vi "C_CRC32.vi"(8 "error in (no error)":errorcluster, 11 "data":u8[](array[numeric]) format="%.0x") -> (0 "error out":errorcluster, 3 "crc32":u32 format="%.0x")   [LabVIEW 2021, in "CANsub_C.lvlib"]
uses:
  CANsub_C.lvlib
  codec_vis/CANsub_Codec.lvlib
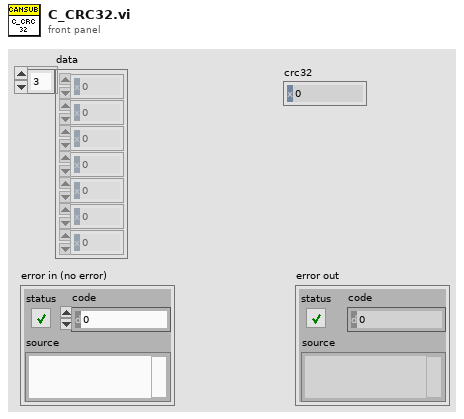
[diagram p1: front panel]
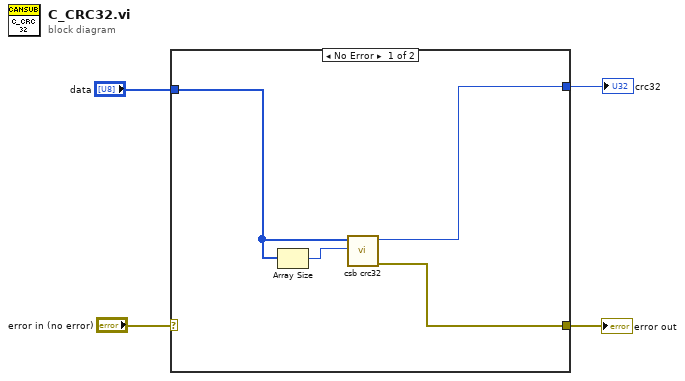
[diagram p0: block diagram]
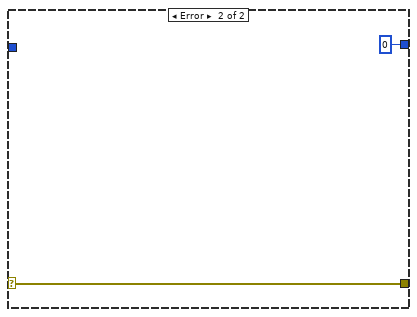
[diagram p2: hidden frame]
diagram:
  n1 = case shown="No Error" "error in (no error)" {
    selector: "error in (no error)" -> [_ w10]
    tunnel: [w8 w10] -> w3
    tunnel: "data" -> [w7 _]
    tunnel: [w5 u32 0 ("function return")] -> w1
    frame No Error {
      n2 = Array Size(array=w7) -> (size(s)=w6:i32)
      n3 = call "csb crc32.vi"("len"=w6, "data"=w7) -> ("error out"=w8:errorcluster, "function return"=w5:u32)  [unwired: 8 in]
    }
    frame Error {
    }
  }
  "crc32" <- w1
  "error out" <- w3
